vi "WriteDataGet.vi"(3 "WriteData":string, 7 "LabVIEW Web Service Request":refnum<class "Web Request.lvclass"> caption="LabVIEW 웹 서비스 요청") -> ()   [LabVIEW 2019]
uses:
  <vilib>/wsapi/Web Request.lvclass
  GlobalValue.vi
panel:
  # "웹 서비스 입력 터미널을 사용하여 웹 서비스 팔레트의 VI를 호출합니다. 팔레트에 접근하지 않아도 되는 경우를 제외하고는 커넥터 팬에서 제거하지 마십시오."
  # "커넥터 팬에 연결된 추가적인 컨트롤은 각각 URL의 입력으로 사용할 수 있습니다. 터미널 모드 출력에 인디케이터를 포함하려면(기본 설정), 역시 커넥터 팬에 연결되어야 합니다."
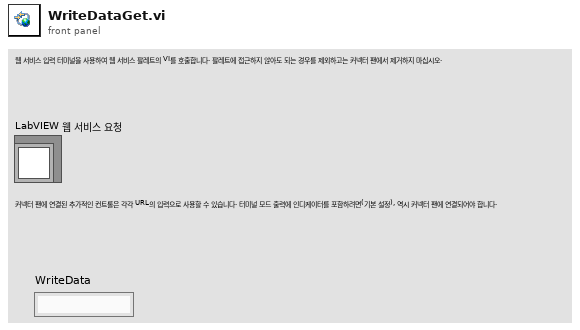
[diagram p1: front panel]
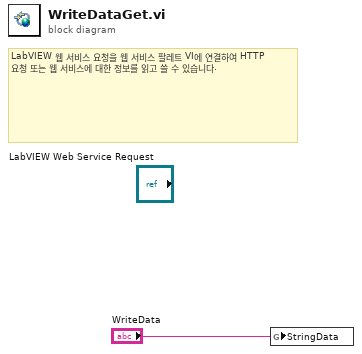
[diagram p0: block diagram]
diagram:
  # "LabVIEW 웹 서비스 요청을 웹 서비스 팔레트 VI에 연결하여 HTTP 요청 또는 웹 서비스에 대한 정보를 읽고 쓸 수 있습니다."
  n1 = global write "GlobalValue.vi" "StringData"("WriteData") -> ()
